vi "Test MQTT-3.1.2-2.vi"(8 "error in (no error)":errorcluster, 11 "Connection Config":refnum<class "Connection.lvclass">) -> (0 "error out":errorcluster, 3 "Connection Config dup":refnum<class "Connection.lvclass">)   [LabVIEW 2013]
uses:
  <vilib>/LabVIEW Open Source Project/MQTT Control Packets/Control Packets/CONNECT/CONNECT.lvclass
  <vilib>/LabVIEW Open Source Project/MQTT Control Packets/Control Packets/ControlPacket/ControlPacket.lvclass
  <vilib>/addons/_JKI Toolkits/Caraya/classes/Test/Test.lvclass
  <vilib>/LabVIEW Open Source Project/MQTT Control Packets/Control Packets/DISCONNECT/DISCONNECT.lvclass
  <vilib>/LabVIEW Open Source Project/MQTT Control Packets/Control Packets/CONNACK/CONNACK.lvclass
  <vilib>/LabVIEW Open Source Project/MQTT Control Packets/Control Packets/CONNACK/Connect Return Code -- enum.ctl
  <vilib>/addons/_JKI Toolkits/Caraya/classes/Assert/Assert.lvclass
  <vilib>/LabVIEW Open Source Project/Connection/Connection/Connection.lvclass
  <vilib>/LabVIEW Open Source Project/MQTT Connection/MQTT_Connection/Connection/Connection.lvclass
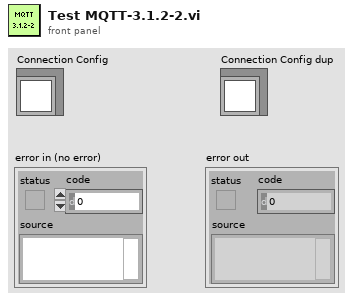
[diagram p1: front panel]
types:
  T1 = typedef "MQTT_Control_Packets.lvlib/CONNACK.lvclass/Connect Return Code -- enum.ctl" = enum16{"Connection accepted", "Unacceptable protocol version", "Identifier Rejected", "Server Unavailable", "Bad Username or Password", "Not Authorized"}
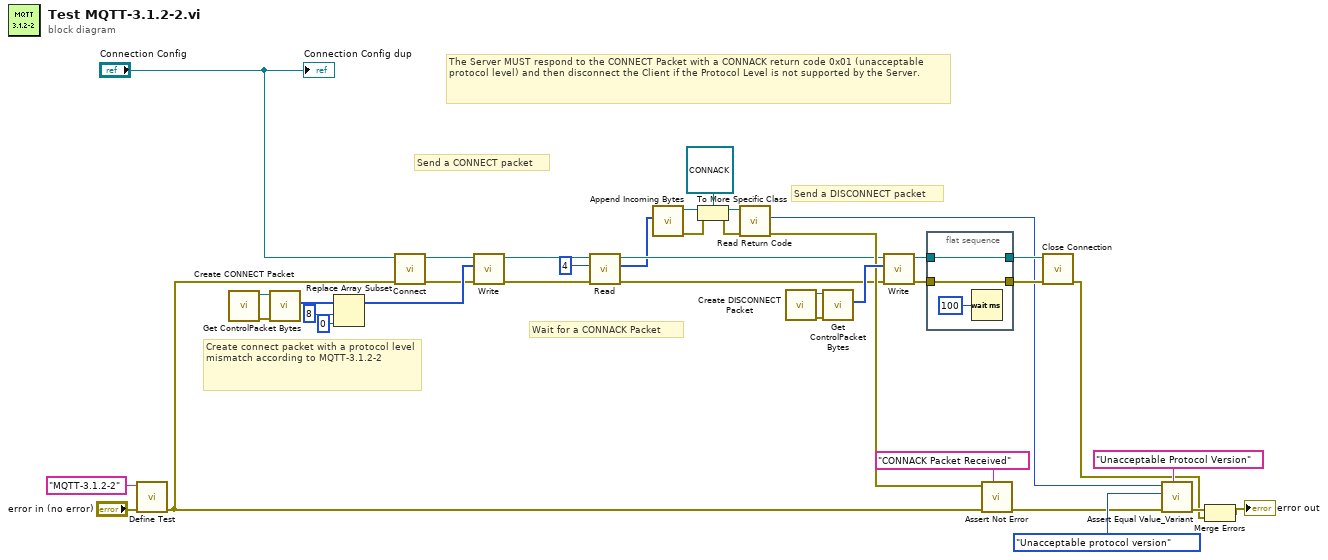
[diagram p0: block diagram]
diagram:
  # "The Server MUST respond to the CONNECT Packet with a CONNACK return code 0x01 (unacceptable protocol level) and then disconnect the Client if the Protocol Level is not supported by the Server."
  # "Send a DISCONNECT packet"
  # "Wait for a CONNACK Packet"
  # "Create connect packet with a protocol level mismatch according to MQTT-3.1.2-2"
  # "Send a CONNECT packet"
  n1 = call <vilib>:"Define Test.vi"("error in (no error)"="error in (no error)", "Label (VI Title)"="MQTT-3.1.2-2") -> ("error out"=w4:errorcluster)  [unwired: 9 in]
  n2 = call <vilib>:"Create CONNECT Packet.vi"() -> ("error out"=w38:errorcluster, "CONNECT"=w39:refnum<class "CONNECT.lvclass">)  [unwired: 9 in, 1 out]
  n3 = call <vilib>:"Get ControlPacket Bytes.vi"("error in (no error)"=w38, "ControlPacket"=w39) -> ("Bytes Stream"=w37:u8[])  [unwired: 6 in, 3 out]
  n4 = Replace Array Subset(array=w37, new element=u8 0 ("new element/subarray"), index=8) -> (w36:u8[])
  n5 = call <vilib>:"Connect.vi"("error in (no error)"=w4, "Connection in"="Connection Config") -> ("error out"=w5:errorcluster, "Connection out"=w6:refnum<class "Connection.lvclass">)  [unwired: 8 in]
  n6 = call <vilib>:"Write.vi"("error in (no error)"=w5, "Bytes"=w36, "Connection in"=w6) -> ("error out"=w9:errorcluster, "Connection"=w10:refnum<class "Connection.lvclass">)  [unwired: 7 in]
  n7 = call <vilib>:"Read.vi"("error in (no error)"=w9, "bytes to read (100)"=4 ("bytes to read"), "TCPConnection in"=w10) -> ("error out"=w3:errorcluster, "Bytes"=w7:u8[], "TCPConnection out"=w8:refnum<class "Connection.lvclass">)  [unwired: 4 in, 2 out]
  n8 = call <vilib>:"Append Incoming Bytes.vi"("Incoming Packets"=w7) -> ("error out"=w12:errorcluster, "ControlPacket"=w21:refnum<class "ControlPacket.lvclass">)  [unwired: 7 in, 2 out]
  n9 = To More Specific Class(target class=refnum<class "CONNACK.lvclass"> refnum ("CONNACK in"), reference=w21, error in=w12) -> (specific class reference=w20:refnum<class "CONNACK.lvclass">, error out=w16:errorcluster)
  n10 = call <vilib>:"Read Return Code.vi"("error in (no error)"=w16, "CONNACK in"=w20) -> ("error out"=w14:errorcluster, "Return Code"=w18:T1)  [unwired: 7 in, 1 out]
  n11 = call <vilib>:"Create DISCONNECT Packet.vi"() -> ("error out"=w29:errorcluster, "DISCONNECT"=w28:refnum<class "DISCONNECT.lvclass">)  [unwired: 9 in, 1 out]
  n12 = call <vilib>:"Get ControlPacket Bytes.vi"("error in (no error)"=w29, "ControlPacket"=w28) -> ("Bytes Stream"=w27:u8[])  [unwired: 6 in, 3 out]
  n13 = call <vilib>:"Write.vi"("error in (no error)"=w3, "Bytes"=w27, "Connection in"=w8) -> ("error out"=w25:errorcluster, "Connection"=w26:refnum<class "Connection.lvclass">)  [unwired: 7 in]
  n14 = flat-sequence {
    tunnel: w26 -> [w42]
    tunnel: [w42] -> w22
    tunnel: [w40] -> w19
    tunnel: w25 -> [w40]
    frame #0 {
      n15 = Wait (ms)(milliseconds to wait=u32 100) -> ()  [unwired: 1 out]
    }
  }
  n16 = call <vilib>:"Assert Not Error.vi"("Label"="CONNACK Packet Received", "error in (no error)"=w4, "Not Error?"=w14) -> ("error out"=w15:errorcluster)  [unwired: 8 in]
  n17 = call <vilib>:"Close Connection.vi"("error in (no error)"=w19, "Connection in"=w22) -> ("error out"=w31:errorcluster)  [unwired: 8 in, 1 out]
  n18 = call <vilib>:"Assert Equal Value_Variant.vi"("Label"="Unacceptable Protocol Version", "error in (no error)"=w15, "Y"=Connect_Return_Code_--_enum."Unacceptable protocol version" ("Return Code"), "X"=w18) -> ("error out"=w34:errorcluster)  [unwired: 7 in]
  n19 = Merge Errors(w34, w31) -> (→"error out":errorcluster)
  "Connection Config dup" <- "Connection Config"
